vi "Cleanup.vi"(8 "error in (no error)":errorcluster, 11 "PanelArray in":refnum<class "ArrayManager.lvclass">) -> (0 "error out":errorcluster, 2 "Events":dbl, 3 "Wait Done":dbl)   [LabVIEW 2020, in "OOPanel.lvlib" / "ArrayManager.lvclass"]
uses:
  ArrayManager.lvclass
  ArrayManager.lvclass/ArrayManager.ctl
  Manager/Manager.lvclass
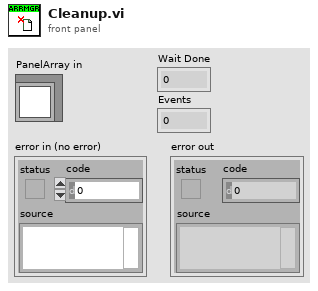
[diagram p1: front panel]
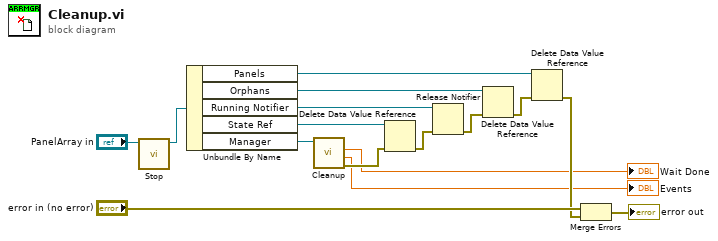
[diagram p0: block diagram]
diagram:
  n1 = call "Stop.vi"("ArrayManager in"="PanelArray in") -> ("ArrayManager out"=w12:refnum<class "ArrayManager.lvclass">)  [unwired: 9 in, 1 out]
  n2 = Unbundle By Name(w12) -> ("Panels"=w6:refnum<data-value>, "Orphans"=w7:refnum<data-value>, "Running Notifier"=w9:refnum<notifier>, "State Ref"=w11:refnum<data-value>, "Manager"=w15:refnum<class "Manager.lvclass">)
  n3 = call "Cleanup.vi"("Manager in"=w15) -> ("error out"=w10:errorcluster, "Events"=→"Events":dbl, "Wait Done"=→"Wait Done":dbl)  [unwired: 8 in]
  n4 = Delete Data Value Reference(data value reference=w11, error in=w10) -> (error out=w8:errorcluster)  [unwired: 1 out]
  n5 = Release Notifier(notifier=w9, error in (no error)=w8) -> (error out=w5:errorcluster)  [unwired: 1 in, 2 out]
  n6 = Delete Data Value Reference(data value reference=w7, error in=w5) -> (error out=w4:errorcluster)  [unwired: 1 out]
  n7 = Delete Data Value Reference(data value reference=w6, error in=w4) -> (error out=w3:errorcluster)  [unwired: 1 out]
  n8 = Merge Errors("error in (no error)", w3) -> (→"error out":errorcluster)
